vi "nevstop-programming-palette - Post-Install Custom Action.vi"(10 "Variant":variant) -> (0 "error out":errorcluster)   [LabVIEW 2017]
uses:
  <vilib>/Palette API/Palette Menu/Public Type Define/Item.ctl
  <vilib>/Palette API/Palette Menu/Public Type Define/Palette type.ctl
  <vilib>/Palette API/Palette Menu/Palette Menu.lvlib
panel:
  out "Array":T1(array[cluster])
  out "concatenated string":string
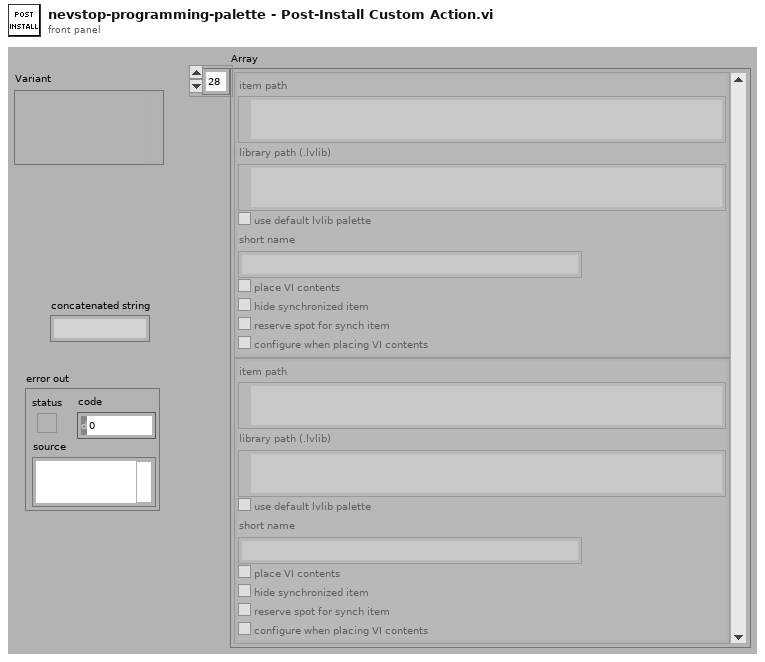
[diagram p1: front panel]
types:
  T1 = cluster{"item path":path, "library path (.lvlib)":path, "use default lvlib palette":bool, "short name":string, "place VI contents":bool, "hide synchronized item":bool, "reserve spot for synch item":bool, "configure when placing VI contents":bool}[]
  T2 = typedef "Palette Menu.lvlib/Item.ctl" = cluster{"item path":path, "library path (.lvlib)":path, "use default lvlib palette":bool, "short name":string, "place VI contents":bool, "hide synchronized item":bool, "reserve spot for synch item":bool, "configure when placing VI contents":bool}
  T3 = cluster{"item path":path, "library path (.lvlib)":path, "use default lvlib palette":bool, "short name":string, "place VI contents":bool, "hide synchronized item":bool, "reserve spot for synch item":bool, "configure when placing VI contents":bool}
  T4 = typedef "Palette Menu.lvlib/Palette type.ctl" = i32
  T5 = typedef "Palette Menu.lvlib/Palette Data.ctl" = cluster{"display name":string, "view format":T6, "palette width":i16, "items":T7, "256 color icon":picture, "B&W color icon":picture, "help information":T8, "palette description":string, "synchronize information":T9}
  T6 = typedef "Palette Menu.lvlib/View Format.ctl" = u16
  T7 = typedef "Palette Menu.lvlib/Items.ctl" = T2[]
  T8 = typedef "Palette Menu.lvlib/Help Info.ctl" = cluster{"help tag":string, "help file path ":path}
  T9 = typedef "Palette Menu.lvlib/Synchronize Info.ctl" = cluster{"synchronize with directory":bool, "synchronize directory path":path}
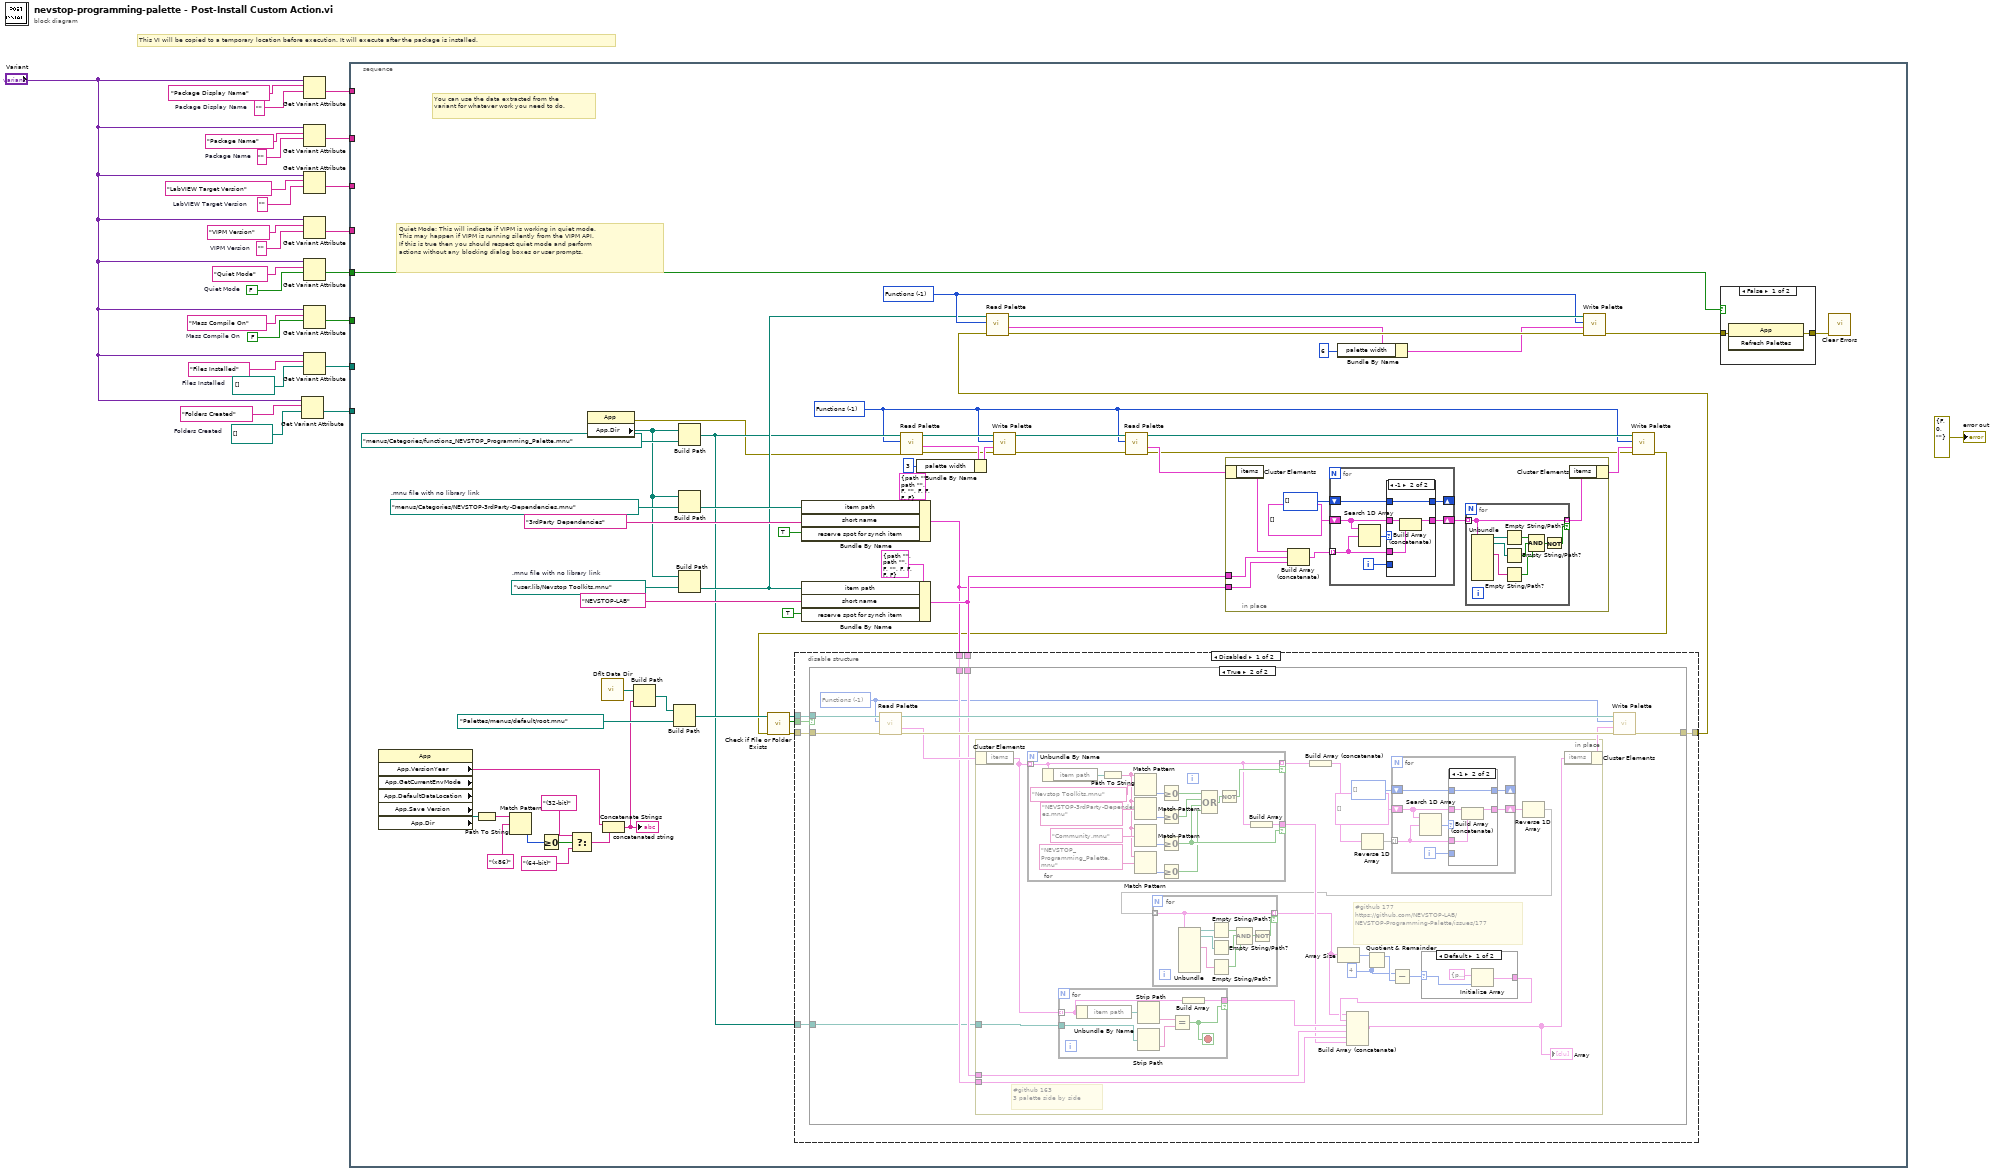
[diagram p0: block diagram]
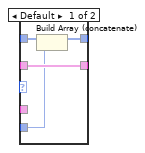
[diagram p4: hidden frame]
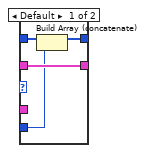
[diagram p6: hidden frame]
diagram:
  w1 = path[] []  # Folders Created
  w2 = path[] []  # Files Installed
  w8 = FALSE  # Mass Compile On
  w9 = ""  # Package Display Name
  w16 = FALSE  # Quiet Mode
  w19 = ""  # VIPM Version
  w21 = ""  # LabVIEW Target Version
  w23 = ""  # Package Name
  # "This VI will be copied to a temporary location before execution. It will execute after the package is installed."
  n1 = Get Variant Attribute(Variant="Variant", name="Folders Created", default value (empty Variant)=w1) -> (value=w6:path[])  [unwired: 1 in, 3 out]
  n2 = Get Variant Attribute(Variant="Variant", name="Package Display Name", default value (empty Variant)=w9) -> (value=w15:string)  [unwired: 1 in, 3 out]
  n3 = Get Variant Attribute(Variant="Variant", name="Package Name", default value (empty Variant)=w23) -> (value=w14:string)  [unwired: 1 in, 3 out]
  n4 = Get Variant Attribute(Variant="Variant", name="LabVIEW Target Version", default value (empty Variant)=w21) -> (value=w13:string)  [unwired: 1 in, 3 out]
  n5 = Get Variant Attribute(Variant="Variant", name="VIPM Version", default value (empty Variant)=w19) -> (value=w12:string)  [unwired: 1 in, 3 out]
  n6 = Get Variant Attribute(Variant="Variant", name="Quiet Mode", default value (empty Variant)=w16) -> (value=w11:bool)  [unwired: 1 in, 3 out]
  n7 = Get Variant Attribute(Variant="Variant", name="Mass Compile On", default value (empty Variant)=w8) -> (value=w10:bool)  [unwired: 1 in, 3 out]
  n8 = Get Variant Attribute(Variant="Variant", name="Files Installed", default value (empty Variant)=w2) -> (value=w5:path[])  [unwired: 1 in, 3 out]
  n9 = stacked-sequence {
    tunnel: w15 -> [_]
    tunnel: w14 -> [_]
    tunnel: w13 -> [_]
    tunnel: w12 -> [_]
    tunnel: w11 -> [w80]
    tunnel: w10 -> [_]
    tunnel: w5 -> [_]
    tunnel: w6 -> [_]
    frame #0 {
      w28 = T4 -1 items=["Functions"=-1, "Controls"=-2] ("palette type")
      w63 = T4 -1 items=["Functions"=-1, "Controls"=-2] ("palette type")
      w71 = path "user.lib/Nevstop Toolkits.mnu"  # .mnu file with no library link
      w75 = path "menus/Categories/NEVSTOP-3rdParty-Dependencies.mnu"  # .mnu file with no library link
      # "Quiet Mode: This will indicate if VIPM is working in quiet mode.\nThis may happen if VIPM is running silently from the VIPM API.\nIf this is true then you should respect quiet mode and perform\nactions without any blocking dialog boxes or user prompts."
      # "You can use the data extracted from the variant for whatever work you need to do."
      n10 = property class="App" props=["App.VersionYear", "App.GetCurrentEnvMode", "App.DefaultDataLocation", "App.Save Version", "App.Dir"]() -> ("App.VersionYear"=w42:string, "App.Dir"=w50:path)  [unwired: 2 in, 5 out]
      n11 = Path To String(path=w50) -> (string=w49:string)
      n12 = Match Pattern(string=w49, regular expression="(x86)") -> (offset past match=w47:i32)  [unwired: 1 in, 3 out]
      n13 = Greater Or Equal To 0?(x=w47) -> (x >= 0?=w46:bool)
      n14 = Select(t="(32-bit)" ("regular expression"), s=w46, f="(64-bit)" ("regular expression")) -> (s? t:f=w43:string)
      n15 = property class="App"() -> (error out=w37:errorcluster, "App.Dir"=w27:path)  [unwired: 2 in, 1 out]
      n16 = call <vilib>:"Dflt Data Dir.vi"() -> ("App:Default Data Directory"=w40:path)
      n17 = Concatenate Strings(w42, w43) -> (w41:string)
      "concatenated string" <- w41
      n18 = Build Path(base path=w40, name or relative path=w41) -> (appended path=w39:path)
      n19 = Build Path(base path=w39, name or relative path=path "Palettes/menus/default/root.mnu") -> (appended path=w55:path)
      n20 = Build Path(base path=w27, name or relative path=path "menus/Categories/functions_NEVSTOP_Programming_Palette.mnu") -> (appended path=w38:path)
      n21 = Build Path(base path=w27, name or relative path=w75) -> (appended path=w79:path)
      n22 = Build Path(base path=w27, name or relative path=w71) -> (appended path=w60:path)
      n23 = Bundle By Name(cluster=T2 {"item path"=path "", "library path (.lvlib)"=path "", "use default lvlib palette"=FALSE, "short name"="", "place VI contents"=FALSE, "hide synchronized item"=FALSE, "reserve spot for synch item"=FALSE, "configure when placing VI contents"=FALSE} ("Items"), "item path"=w79, "short name"="3rdParty Dependencies" ("short name (standard)"), "reserve spot for synch item"=TRUE) -> (w57:T2)
      n24 = Bundle By Name(cluster=T2 {"item path"=path "", "library path (.lvlib)"=path "", "use default lvlib palette"=FALSE, "short name"="", "place VI contents"=FALSE, "hide synchronized item"=FALSE, "reserve spot for synch item"=FALSE, "configure when placing VI contents"=FALSE} ("Items"), "item path"=w60, "short name"="NEVSTOP-LAB" ("short name (standard)"), "reserve spot for synch item"=TRUE) -> (w59:T2)
      n25 = call <vilib>:"Read Palette.vi"("error in (no error)"=w37, "palette type"=w28, "palette path"=w38) -> ("error out"=w34:errorcluster, "palette data"=w72:T5, "duplicate palette path"=w33:path)  [unwired: 1 in, 5 out]
      n26 = Bundle By Name(cluster=w72, "palette width"=i16 3) -> (w35:T5)
      n27 = call <vilib>:"Write Palette.vi"("error in (no error)"=w34, "palette data"=w35, "palette type"=w28, "palette path"=w33) -> ("error out"=w32:errorcluster)  [unwired: 1 in, 6 out]
      n28 = call <vilib>:"Read Palette.vi"("error in (no error)"=w32, "palette type"=w28, "palette path"=w33) -> ("error out"=w30:errorcluster, "palette data"=w31:T5, "duplicate palette path"=w29:path)  [unwired: 1 in, 5 out]
      n29 = in-place {
        in-place-border: w57 -> [w177]
        in-place-border: w59 -> [w178]
        n30 = in-place-cluster #1(w31) -> ("items"=w176:T7)
        n31 = Build Array (concatenate)(w176, w178, w177) -> (w179:T7)
        n32 = for {
          tunnel: w179 -> [w196] mode=indexing
          shift-right: [w195] -> w174
          shift-left: T2[] [] -> [w194]
          shift-right: [w192] -> _
          shift-left: i32[] [] -> [w191]
          i -> [w193]
          n33 = Search 1D Array(1D array=w194, element=w196) -> (index of element=w197:i32)  [unwired: 1 in]
          n34 = case shown="-1" w197 {
            tunnel: w196 -> [_ w205]
            tunnel: [w201 w203] -> w195
            tunnel: w194 -> [w201 w204]
            tunnel: w193 -> [w198 _]
            tunnel: [w199 w202] -> w192
            tunnel: w191 -> [w200 w202]
            frame Default {
              n35 = Build Array (concatenate)(w200, w198) -> (w199:i32[])
            }
            frame -1 {
              n36 = Build Array (concatenate)(w204, w205) -> (w203:T2[])
            }
          }
        }
        n37 = for {
          tunnel: [w190] -> w175 mode=indexing if=w182
          tunnel: w174 -> [w190] mode=indexing
          n38 = Unbundle(w190) -> ("item path"=w189:path, "library path (.lvlib)"=w187:path, "short name"=w188:string)  [unwired: 5 out]
          n39 = Empty String/Path?(string/path=w189) -> (empty?=w186:bool)
          n40 = Empty String/Path?(string/path=w187) -> (empty?=w185:bool)
          n41 = Empty String/Path?(string/path=w188) -> (empty?=w184:bool)
          n42 = Compound Arithmetic op=AND(w186, w185, w184) -> (w183:bool)
          n43 = Not(x=w183) -> (.not. x?=w182:bool)
        }
        n44 = in-place-cluster #1("items"=w175) -> (w73:T5)
      }
      n45 = call <vilib>:"Write Palette.vi"("error in (no error)"=w30, "palette data"=w73, "palette type"=w28, "palette path"=w29) -> ("error out"=w53:errorcluster)  [unwired: 1 in, 6 out]
      n46 = call <vilib>:"Check if File or Folder Exists.vi"("error in (no error)"=w53, "path"=w55) -> ("error out"=w52:errorcluster, "file or folder exists?"=w51:bool, "dup path"=w54:path)  [unwired: 7 in]
      n47 = disable-structure shown="Disabled" {
        disable-tunnel: w59 -> [w88 _]
        disable-tunnel: [w87 w173] -> w58
        disable-tunnel: w57 -> [w86 _]
        disable-tunnel: w54 -> [w85 _]
        disable-tunnel: w52 -> [w84 w173]
        disable-tunnel: w51 -> [w83 _]
        disable-tunnel: w38 -> [w82 _]
        frame Disabled {
          n48 = case shown="True" w83 {
            tunnel: w88 -> [_ w96]
            tunnel: [w89 w95] -> w87
            tunnel: w86 -> [_ w94]
            tunnel: w85 -> [_ w93]
            tunnel: w84 -> [w89 w92]
            tunnel: w82 -> [_ w91]
            frame False {
            }
            frame True {
              w90 = T4 -1 items=["Functions"=-1, "Controls"=-2] ("palette type")
              n49 = call <vilib>:"Read Palette.vi"("error in (no error)"=w92, "palette type"=w90, "palette path"=w93) -> ("error out"=w100:errorcluster, "palette data"=w98:T5, "duplicate palette path"=w99:path)  [unwired: 1 in, 5 out]
              n50 = in-place {
                in-place-border: w96 -> [w110]
                in-place-border: w94 -> [w111]
                in-place-border: w91 -> [w116]
                w106 = 4 ("y")
                # "#github 177\nhttps://github.com/NEVSTOP-LAB/NEVSTOP-Programming-Palette/issues/177"
                # "#github 163\n3 palette side by side"
                n51 = in-place-cluster #2(w98) -> ("items"=w114:T7)
                n52 = for {
                  tunnel: w114 -> [w130] mode=indexing
                  tunnel: [w130] -> w113 mode=indexing if=w134
                  tunnel: [w129] -> w109 if=w128
                  n53 = Unbundle By Name(w130) -> ("item path"=w141:path)
                  n54 = Path To String(path=w141) -> (string=w125:string)
                  n55 = Match Pattern(string=w125, regular expression="Nevstop Toolkits.mnu" ("y")) -> (offset past match=w138:i32)  [unwired: 1 in, 3 out]
                  n56 = Match Pattern(string=w125, regular expression="NEVSTOP-3rdParty-Dependencies.mnu" ("y")) -> (offset past match=w137:i32)  [unwired: 1 in, 3 out]
                  n57 = Match Pattern(string=w125, regular expression="Community.mnu" ("y")) -> (offset past match=w133:i32)  [unwired: 1 in, 3 out]
                  n58 = Match Pattern(string=w125, regular expression="NEVSTOP_Programming_Palette.mnu" ("y")) -> (offset past match=w126:i32)  [unwired: 1 in, 3 out]
                  n59 = Greater Or Equal To 0?(x=w138) -> (x >= 0?=w135:bool)
                  n60 = Greater Or Equal To 0?(x=w137) -> (x >= 0?=w136:bool)
                  n61 = Greater Or Equal To 0?(x=w133) -> (x >= 0?=w128:bool)
                  n62 = Greater Or Equal To 0?(x=w126) -> (x >= 0?=w124:bool)
                  n63 = Compound Arithmetic op=OR(w135, w136, w128, w124) -> (w140:bool)
                  n64 = Not(x=w140) -> (.not. x?=w134:bool)
                  n65 = Build Array(w130) -> (w129:T2[])
                }
                n66 = for {
                  tunnel: w114 -> [w153] mode=indexing
                  tunnel: w116 -> [w154]
                  tunnel: [w152] -> w112 if=w151
                  stop <- w151 stop-if-true
                  n67 = Unbundle By Name(w153) -> ("item path"=w156:path)
                  n68 = Strip Path(path=w156) -> (name=w157:string)  [unwired: 1 out]
                  n69 = Strip Path(path=w154) -> (name=w155:string)  [unwired: 1 out]
                  n70 = Equal?(x=w157, y=w155) -> (x = y?=w151:bool)
                  n71 = Build Array(w153) -> (w152:T2[])
                }
                n72 = Build Array (concatenate)(w113) -> (w120:T2[])
                n73 = Reverse 1D Array(array=w120) -> (reversed array=w115:T2[])
                n74 = for {
                  tunnel: w115 -> [w163] mode=indexing
                  shift-right: [w162] -> w117
                  shift-left: T2[] [] -> [w161]
                  shift-right: [w159] -> _
                  shift-left: i32[] [] -> [w158]
                  i -> [w160]
                  n75 = Search 1D Array(1D array=w161, element=w163) -> (index of element=w164:i32)  [unwired: 1 in]
                  n76 = case shown="-1" w164 {
                    tunnel: w163 -> [_ w172]
                    tunnel: [w168 w170] -> w162
                    tunnel: w161 -> [w168 w171]
                    tunnel: w160 -> [w165 _]
                    tunnel: [w166 w169] -> w159
                    tunnel: w158 -> [w167 w169]
                    frame Default {
                      n77 = Build Array (concatenate)(w167, w165) -> (w166:i32[])
                    }
                    frame -1 {
                      n78 = Build Array (concatenate)(w171, w172) -> (w170:T2[])
                    }
                  }
                }
                n79 = Reverse 1D Array(array=w117) -> (reversed array=w103:T2[])
                n80 = for {
                  tunnel: [w150] -> w102 mode=indexing if=w142
                  tunnel: w103 -> [w150] mode=indexing
                  n81 = Unbundle(w150) -> ("item path"=w149:path, "library path (.lvlib)"=w147:path, "short name"=w148:string)  [unwired: 5 out]
                  n82 = Empty String/Path?(string/path=w149) -> (empty?=w146:bool)
                  n83 = Empty String/Path?(string/path=w147) -> (empty?=w145:bool)
                  n84 = Empty String/Path?(string/path=w148) -> (empty?=w144:bool)
                  n85 = Compound Arithmetic op=AND(w146, w145, w144) -> (w143:bool)
                  n86 = Not(x=w143) -> (.not. x?=w142:bool)
                }
                n87 = Array Size(array=w102) -> (size(s)=w108:i32)
                n88 = Quotient & Remainder(x=w108, y=w106) -> (x-y*floor(x/y)=w107:i32)  [unwired: 1 out]
                n89 = Subtract(x=w106, y=w107) -> (x-y=w105:i32)
                n90 = case shown="Default" w105 {
                  selector: w105 -> [w122 _]
                  tunnel: [w121 _] -> w104
                  frame Default {
                    n91 = Initialize Array(T3 {"item path"=path "", "library path (.lvlib)"=path "", "use default lvlib palette"=FALSE, "short name"="", "place VI contents"=FALSE, "hide synchronized item"=FALSE, "reserve spot for synch item"=FALSE, "configure when placing VI contents"=FALSE} ("Items"), w122) -> (w121:T1)
                  }
                  frame 0 {
                  }
                }
                n92 = Build Array (concatenate)(w102, w104, w112, w110, w111, w109) -> (w101:T2[])
                "Array" <- w101
                n93 = in-place-cluster #2("items"=w101) -> (w97:T5)
              }
              n94 = call <vilib>:"Write Palette.vi"("error in (no error)"=w100, "palette data"=w97, "palette type"=w90, "palette path"=w99) -> ("error out"=w95:errorcluster)  [unwired: 1 in, 6 out]
            }
          }
        }
        frame Enabled {
        }
      }
      n95 = call <vilib>:"Read Palette.vi"("error in (no error)"=w58, "palette type"=w63, "palette path"=w60) -> ("error out"=w67:errorcluster, "palette data"=w66:T5, "duplicate palette path"=w64:path)  [unwired: 1 in, 5 out]
      n96 = Bundle By Name(cluster=w66, "palette width"=i16 6) -> (w65:T5)
      n97 = call <vilib>:"Write Palette.vi"("error in (no error)"=w67, "palette data"=w65, "palette type"=w63, "palette path"=w64) -> ("error out"=w61:errorcluster)  [unwired: 1 in, 6 out]
      n98 = case shown="False" w80 {
        tunnel: [w207 w208] -> w81
        tunnel: w61 -> [w206 w208]
        frame False {
          n99 = invoke class="App" method="Refresh Palettes"(error in=w206) -> (error out=w207:errorcluster)  [unwired: 2 in, 2 out]
        }
        frame True {
        }
      }
      n100 = call <vilib>:"Clear Errors.vi"("error in (no error)"=w81) -> ()  [unwired: 5 in, 2 out]
    }
  }
  "error out" <- errorcluster {"status"=FALSE, "code"=0, "source"=""} ("error out")
